vi "VIH Dialog - Quick Tips.vi"(10 "Tip#":i32=-1) -> (2 "Tip# out":i32=-1, 3 "ShowAtStartup out":bool)   [LabVIEW 2014]
doc: "::: VI Helpeks :::\nCopyright (c) 2000-2026 Konstantin Shifershteyn. All rights reserved."
uses:
  <vilib>/Platform/browser.llb/Open URL in Default Browser (string).vi
  _VIH Support Library.llb/VIH Utility - APP - Is Value Changed (U32).vi
  <vilib>/Utility/cursorutil.llb/Set Cursor (Icon Pict).vi
panel:
  out "counter":string
  in  "%First":bool
  out "Tip Title":string
  in  "%Next":bool
  in  "%Prev":bool
  in  "%OK":bool
  in  "ShowAtStartup":bool=TRUE caption="Don't show anymore"
  out "Tip Text":string
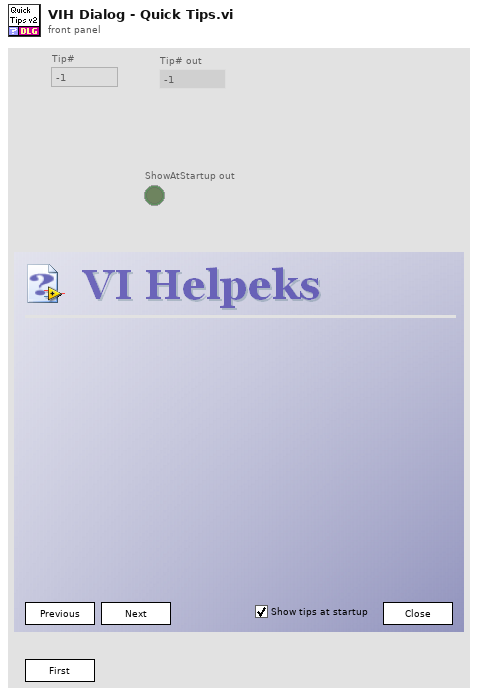
[diagram p1: front panel]
types:
  T1 = typedef "eventvkey.ctl" = enum16{"ASCII", "Enter", "Return", "Shift", "Ctrl", "Alt", "Cmd", "Opt", "Caps", "NumLock", "Clear", "Break", "Up", "Down", "Left", "Right", "Insert", "Delete", "Home", "End", "PageUp", "PageDown", "Escape", "Help", "Pause", "ScrollLock", "F1", "F2", "F3", "F4", "F5", "F6", "F7", "F8", "F9", "F10", "F11", "F12", "F13", "F14", "F15", "F16", "F17", "F18", "F19", "F20", "F21", "F22", "F23", "F24", "Play", "VolumeUp", "VolumeDown", "Mute", "Two Byte Char"}
  T2 = cluster{"Shift":bool, "Ctrl":bool, "Alt":bool, "Cmd":bool, "Opt":bool}
  T3 = typedef "LVPoint32TypeDef.ctl" = cluster{"Horizontal":i32, "Vertical":i32}
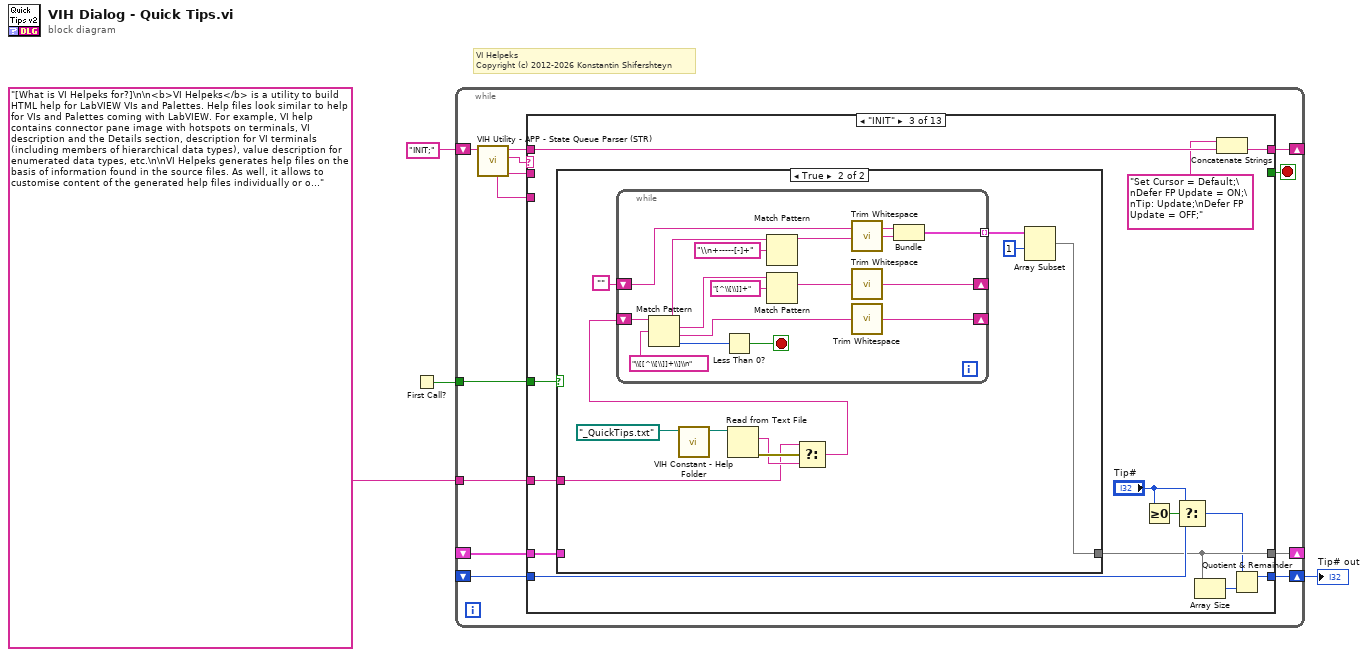
[diagram p0: block diagram]
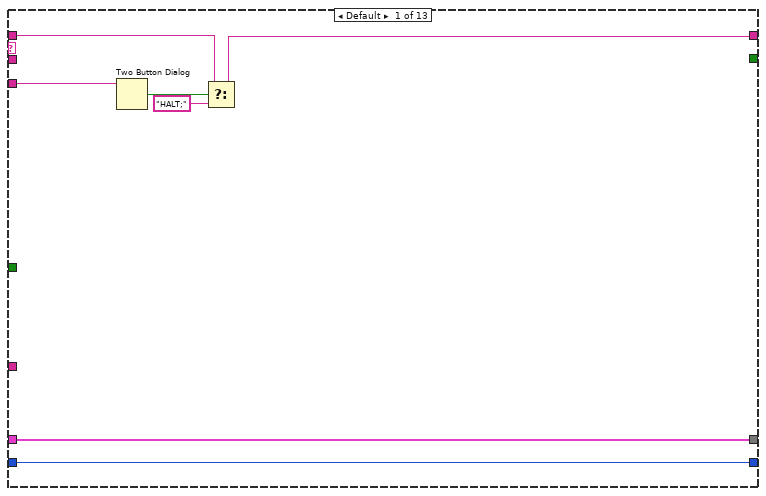
[diagram p2: hidden frame]
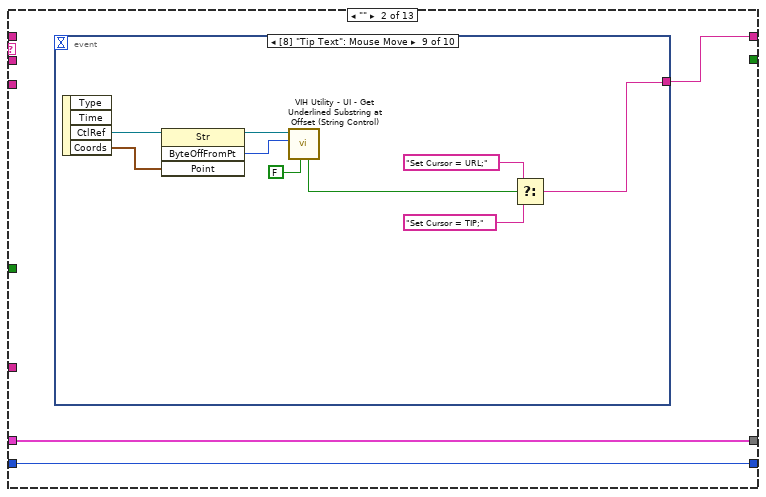
[diagram p3: hidden frame]
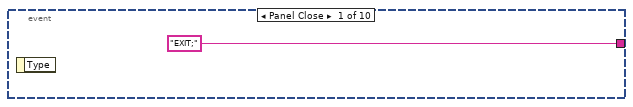
[diagram p4: hidden frame]
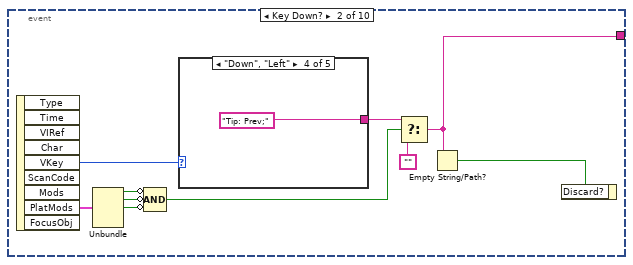
[diagram p5: hidden frame]
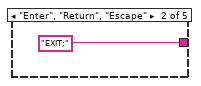
[diagram p7: hidden frame]
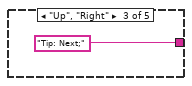
[diagram p8: hidden frame]
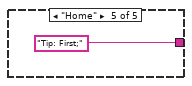
[diagram p9: hidden frame]
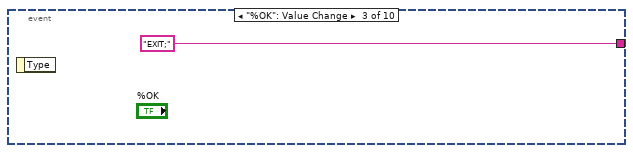
[diagram p10: hidden frame]
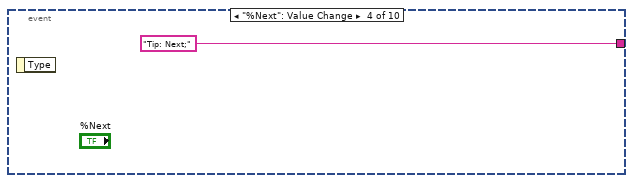
[diagram p11: hidden frame]
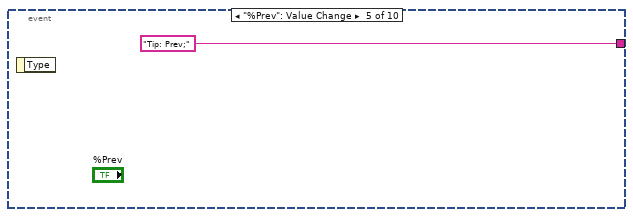
[diagram p12: hidden frame]
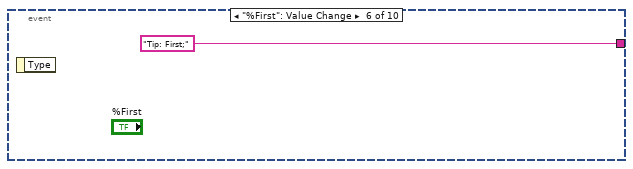
[diagram p13: hidden frame]
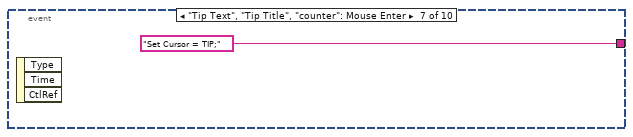
[diagram p14: hidden frame]
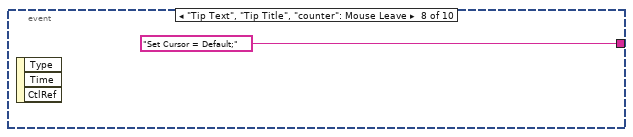
[diagram p15: hidden frame]
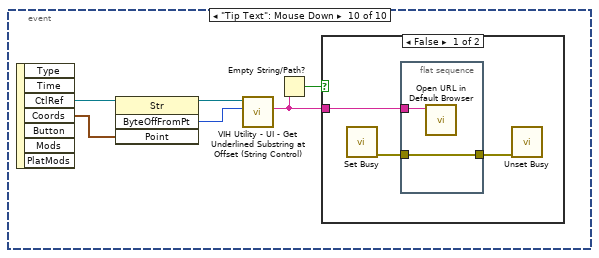
[diagram p16: hidden frame]
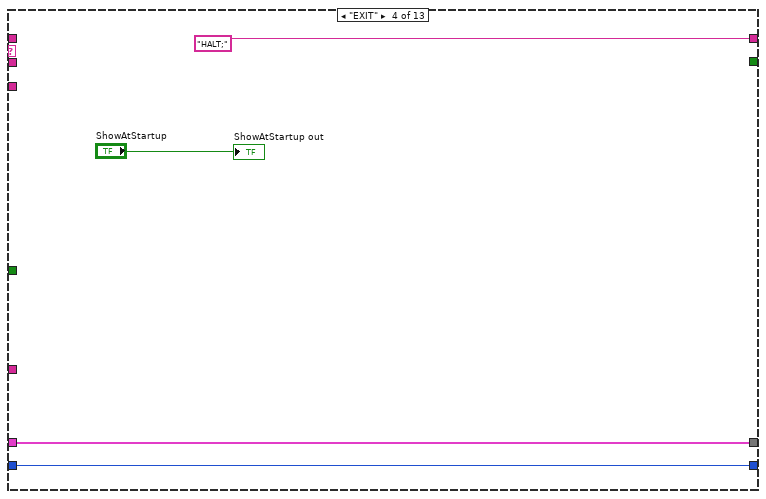
[diagram p19: hidden frame]
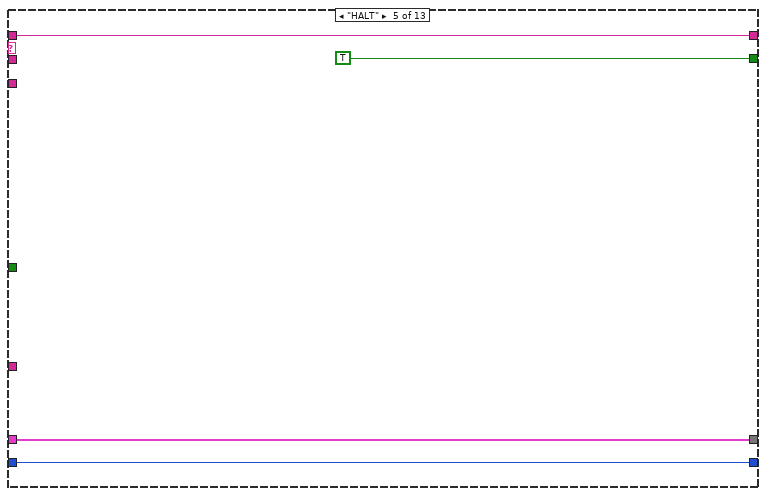
[diagram p20: hidden frame]
diagram:
  # "VI Helpeks\nCopyright (c) 2012-2026 Konstantin Shifershteyn"
  n1 = First Call?() -> (First Call?: T/F=w3:bool)
  n2 = while {
    shift-right: [w13] -> _
    shift-left: "INIT;" -> [w17]
    shift-right: [w11] -> _
    shift-left: _ -> [w10]
    shift-right: [w9] -> w1
    shift-left: _ -> [w8]
    tunnel: w3 -> [w7]
    tunnel: "[What is VI Helpeks for?]\n\n<b>VI Helpeks</b> is a utility to build HTML help for LabVIEW VIs and Palettes. Help files look similar to help for VIs and Palettes coming with LabVIEW. For example, VI help contains connector pane image with hotspots on terminals, VI description and the Details section, description for VI terminals (including members of hierarchical data types), value description for enumerated data types, etc.\n\nVI Helpeks generates help files on the basis of information found in the source files. As well, it allows to customise content of the generated help files individually or on group basis.\n\n------------------------\n\n[Help and Examples]\n\nTo learn overall concept of VI Helpeks, select <b>Help >> Open Help</b> menu.\n\nUse LabVIEW <b>Context Help</b> to get information on controls or indicators in the main VI Helpeks window as well as in any dialog. Context help might contain not only help on using a control or indicator but also relevant background information.\n\nVI Helpeks comes with a few example projects that demonstrate its capabilities and some details of use. Use <b>Help >> Open Example Project</b> menu to open an example project. When you open a project, build it with the <b>Build >> Build Help for All</b> menu. After the build completes, you can review generated help in your default browser.\n\n------------------------\n\n[A few GUI tips]\n\nShortcut menus are available for the Project Tree in the main VI Helpeks window as well as for controls in many dialog windows.\n\nMultiple items selection is allowed in tree and listbox controls in the main VI Helpeks window and dialog windows.\n\nYou can resize the main VI Helpeks window and some of dialog windows.\n\n------------------------\n\n[Build help]\n\nBuild help for all project files with <b>Build >> Build Help for All</b> menu.\n\nYou can build help for project files individually. For this, highlight desired file(s) in the Project Tree, activate shortcut menu and select either <b>Build Help (selected only)</b> or <b>Build Help (selected & underlying)</b>. The last option is for Palette menus, it will build help for the selected Palette and all its sub-palettes and VIs recursively.\n\nYou can build help for project files in a group. For this, highlight desired group(s) in the Project Tree, activate shortcut menu and select <b>Build help for underlying files</b>. Help will be built for all underlying files recursively.\n\n------------------------\n\n[Build Destination folder]\n\nWhen you create a new project or open an example project, destination folder for output files is set beneath the default temporary directory on your computer. If you want to change the target folder, select either <b>Help Project</b> or <b>Project Files</b> item in the Project Tree, select the <b>Target Paths</b> category and specify the desired path in the <b>Build Root Folder</b> control.\n\n------------------------\n\n[Open built help files]\n\nIn order to open an output help file, highlight the respective source file in the Project Tree, activate shortcut menu and select <b>Open Output Help File</b>. Also, you can do this using the main menu (<b>Project >> Open Output Help File</b>).\n\nVI Helpeks opens help files in your default browser.\n\n------------------------\n\n[Project types]\n\nVI Helpeks generates help files on the basis of template files. Appearance and behavior of output help files are defined by the set of template files used in a project. When you create a new project, its Master Rule is configured to use template files relevant for the project type you choose:\n*** <b>Default</b> project type is for generating pure frameless HTML files.\n*** <b>JavaScript based</b> project type is for generating HTML files that utilize JavaScripts for additional features.\n\nYou can easy reconfigure the Master Rule of your project for a desired project type through <b>File >> Change project type</b> menu.\n\n-----------------------\n\n[Images in help files]\n\nVI Helpeks creates help files with images that look the same as you see them in the LabVIEW version it's running. It does not use any template images for control terminals, but retrieves actual images from LabVIEW (including typedefs and members of hierarchical data structures). VI connector pane images look the same as in the LabVIEW Context Help.\n\n-----------------------\n\n[Hotspots in VI connector pane images]\n\nA help file generated for a VI contains connector pane image with hotspots at VI terminals. If you click a terminal name in the connector pane image, you are navigated to the respective control description in the help file.\n\nSimilarly, when you open <b>VI Terminals</b> dialog, you can click a VI terminal name in the connector pane image in order to select respective control (with its descendants, optionaly) in the Control Tree. Use Context Help for controls in this dialog to get more information.\n\n------------------------\n\n[Source VI state]\n\nSource VIs, for which you are going to build help, are not restricted to be in the idle state. VI Helpeks can build help for running VIs. As well, it can build help for locked and password protected VIs.\n\n------------------------\n\n[Compiled HTML Help (.CHM)]\n\nVI Helpeks doesn't create compiled help files (CHM) by itself. Instead, it creates HTML Help Project (HHP) for <b>HTML Help Workshop</b> by Microsoft, which can compile CHM files for you.\n\nSelect <b>Build >> Compiled HTML Help</b> menu to run a utility that helps you to create compiled help files.\n\nIf you don't have <b>HTML Help Workshop</b> installed, you can download it at Microsoft website for free:\n<link>http://msdn.microsoft.com/en-us/library/ms669985.aspx</link>\n" -> [w6]
    stop <- w12 stop-if-true
    n3 = call "VIH Utility - APP - State Queue Parser (STR).vi"("input queue"=w17) -> ("state parameters"=w5:string, "state"=w16:string, "remained queue"=w14:string, "complete state specifier"=w15:string)  [unwired: 5 in]
    n4 = case shown="\"INIT\"" w16 {
      tunnel: w15 -> [w24 _ _ _ _ _ _ _ _ _ _ _ _]
      tunnel: w14 -> [w22 _ w81 _ w116 w119 w127 w134 w142 w153 w161 w164 w174]
      tunnel: [w21 w27 w74 "HALT;" w116 w119 w127 w134 w142 w153 w155 w163 w173] -> w13
      tunnel: [_ _ _ _ TRUE _ _ _ _ _ _ _ _] -> w12
      tunnel: [w19 w26 w75 w110 w114 w118 w126 w133 w141 w146 w160 w171 w176] -> w11
      tunnel: w10 -> [w19 w26 w79 w110 w114 w118 w126 w133 w141 w146 w160 w171 w176]
      tunnel: [w18 w25 w70 w109 w113 w117 w125 w132 w140 w148 w158 w167 0] -> w9
      tunnel: w8 -> [w18 w25 w76 w109 w113 w117 w125 w132 w140 w148 w159 w170 _]
      tunnel: w7 -> [_ _ w80 _ _ _ _ _ _ _ _ _ _]
      tunnel: w6 -> [_ _ w78 _ _ _ _ _ _ _ _ _ _]
      tunnel: w5 -> [_ _ _ _ _ _ w120 w131 _ _ _ _ _]
      frame Default {
        n5 = Two Button Dialog(message=w24) -> (T button?=w23:bool)  [unwired: 2 in]
        n6 = Select(t=w22, s=w23, f="HALT;") -> (s? t:f=w21:string)
      }
      frame "" {
        n7 = event shown="[8] \"Tip Text\": Mouse Move" {
          selector: _ -> [_ _ _ _ _ _ _ _ _ _]
          dyn-events: _ -> [_ _ _ _ _ _ _ _ _ _]
          timeout: _ -> [_ _ _ _ _ _ _ _ _ _]
          tunnel: ["EXIT;" w30 "EXIT;" "Tip: Next;" "Tip: Prev;" "Tip: First;" "Set Cursor = TIP;" "Set Cursor = Default;" w53 _] -> w27
          event Panel Close {
            n8 = event-data() -> ()  [unwired: 1 in, 1 out]
          }
          event Key Down? {
            n9 = event-data() -> ("VKey"=w33:T1, "PlatMods"=w38:T2)  [unwired: 1 in, 7 out]
            n10 = Unbundle(w38) -> ("Shift"=w37:bool, "Ctrl"=w36:bool, "Alt"=w35:bool)  [unwired: 2 out]
            n11 = Compound Arithmetic op=AND(invert w37, invert w36, invert w35) -> (w34:bool)
            n12 = case shown="\"Down\", \"Left\"" w33 {
              tunnel: [_ "EXIT;" "Tip: Next;" "Tip: Prev;" "Tip: First;"] -> w32
              frame Default {
              }
              frame "Enter", "Return", "Escape" {
              }
              frame "Up", "Right" {
              }
              frame "Down", "Left" {
              }
              frame "Home" {
              }
            }
            n13 = Select(t=w32, s=w34, f="") -> (s? t:f=w30:string)
            n14 = Empty String/Path?(string/path=w30) -> (empty?=w31:bool)
            n15 = event-data("Discard?"=w31) -> ()  [unwired: 1 in, 1 out]
          }
          event "%OK": Value Change {
            n16 = event-data() -> ()  [unwired: 1 in, 1 out]
          }
          event "%Next": Value Change {
            n17 = event-data() -> ()  [unwired: 1 in, 1 out]
          }
          event "%Prev": Value Change {
            n18 = event-data() -> ()  [unwired: 1 in, 1 out]
          }
          event "%First": Value Change {
            n19 = event-data() -> ()  [unwired: 1 in, 1 out]
          }
          event "Tip Text", "Tip Title", "counter": Mouse Enter {
            n20 = event-data() -> ()  [unwired: 1 in, 3 out]
          }
          event "Tip Text", "Tip Title", "counter": Mouse Leave {
            n21 = event-data() -> ()  [unwired: 1 in, 3 out]
          }
          event "Tip Text": Mouse Move {
            n22 = event-data() -> ("CtlRef"=w56:refnum<vi>, "Coords"=w57:T3)  [unwired: 1 in, 2 out]
            n23 = invoke class="Str" method="ByteOffFromPt"(reference=w56, "Point"=w57) -> (reference out=w55:refnum<vi>, "ByteOffFromPt"=w54:i32)  [unwired: 2 in, 2 out]
            n24 = call "VIH Utility - UI - Get Underlined Substring at Offset (String Control).vi"("Get string (T)"=FALSE, "Offset"=w54, "Str Refnum"=w55) -> ("active"=w51:bool)  [unwired: 4 in, 4 out]
            n25 = Select(t="Set Cursor = URL;", s=w51, f="Set Cursor = TIP;") -> (s? t:f=w53:string)
          }
          event "Tip Text": Mouse Down {
            n26 = event-data() -> ("CtlRef"=w62:refnum<vi>, "Coords"=w63:T3)  [unwired: 1 in, 5 out]
            n27 = invoke class="Str" method="ByteOffFromPt"(reference=w62, "Point"=w63) -> (reference out=w61:refnum<vi>, "ByteOffFromPt"=w60:i32)  [unwired: 2 in, 2 out]
            n28 = call "VIH Utility - UI - Get Underlined Substring at Offset (String Control).vi"("Offset"=w60, "Str Refnum"=w61) -> ("String"=w59:string)  [unwired: 5 in, 4 out]
            n29 = Empty String/Path?(string/path=w59) -> (empty?=w58:bool)
            n30 = case shown="False" w58 {
              tunnel: w59 -> [w66 _]
              frame False {
                n31 = call <vilib>:"Set Busy.vi"() -> ("error out"=w64:errorcluster)  [unwired: 10 in, 1 out]
                n32 = flat-sequence {
                  tunnel: w66 -> [w68]
                  tunnel: [w67] -> w65
                  tunnel: w64 -> [w67]
                  frame #0 {
                    n33 = call-poly <vilib>:"Open URL in Default Browser.vi"("URL"=w68) -> ()  [unwired: 5 in, 2 out]
                  }
                }
                n34 = call <vilib>:"Unset Busy.vi"("error in (no error)"=w65) -> ()  [unwired: 10 in, 1 out]
              }
              frame True {
              }
            }
          }
        }
      }
      frame "INIT" {
        n35 = case shown="True" w80 {
          tunnel: [w82 w85] -> w75
          tunnel: w79 -> [w82 _]
          tunnel: w78 -> [_ w87]
          frame False {
          }
          frame True {
            n36 = call "VIH Constant - Help Folder.vi"("append path"=path "_QuickTips.txt" ("Path")) -> ("Help path"=w84:path)  [unwired: 10 in]
            n37 = Read from Text File(file (use dialog)=w84) -> (text=w88:string, error out=w89:errorcluster)  [unwired: 3 in, 2 out]
            n38 = Select(t=w87, s=w89, f=w88) -> (s? t:f=w86:string)
            n39 = while {
              shift-right: [w97] -> _
              shift-left: w86 -> [w108]
              shift-right: [w98] -> _
              shift-left: "" -> [w101]
              tunnel: [w100] -> w91 mode=indexing
              stop <- w105 stop-if-true
              n40 = Match Pattern(string=w108, regular expression="\\[[^\\[\\]]+\\]\\n") -> (before substring=w93:string, match substring=w95:string, after substring=w104:string, offset past match=w106:i32)  [unwired: 1 in]
              n41 = Less Than 0?(x=w106) -> (x < 0?=w105:bool)
              n42 = Match Pattern(string=w93, regular expression="\\n+-----[-]+") -> (before substring=w94:string)  [unwired: 1 in, 3 out]
              n43 = Match Pattern(string=w95, regular expression="[^\\[\\]]+") -> (match substring=w102:string)  [unwired: 1 in, 3 out]
              n44 = call <vilib>:"Trim Whitespace.vi"("string"=w94) -> ("trimmed string"=w99:string)  [unwired: 1 in]
              n45 = call <vilib>:"Trim Whitespace.vi"("string"=w102) -> ("trimmed string"=w98:string)  [unwired: 1 in]
              n46 = call <vilib>:"Trim Whitespace.vi"("string"=w104) -> ("trimmed string"=w97:string)  [unwired: 1 in]
              n47 = Bundle(w101, "trimmed string"=w99) -> (w100:cluster{string, "trimmed string":string})  [unwired: 1 in]
            }
            n48 = Array Subset(array=w91, index=1) -> (w85:cluster{string, "trimmed string":string}[])  [unwired: 1 in]
          }
        }
        n49 = Greater Or Equal To 0?(x="Tip#") -> (x >= 0?=w77:bool)
        n50 = Select(t="Tip#", s=w77, f=w76) -> (s? t:f=w69:i32)
        n51 = Array Size(array=w75) -> (size(s)=w71:i32)
        n52 = Concatenate Strings("Set Cursor = Default;\nDefer FP Update = ON;\nTip: Update;\nDefer FP Update = OFF;", w81) -> (w74:string)
        n53 = Quotient & Remainder(x=w69, y=w71) -> (x-y*floor(x/y)=w70:i32)  [unwired: 1 out]
      }
      frame "EXIT" {
        "ShowAtStartup out" <- "ShowAtStartup"
      }
      frame "HALT" {
      }
      frame "------------------------------ 1" {
      }
      frame "Defer FP Update" {
        n54 = To Upper Case(1:w120) -> (0:w123:string)
        n55 = Equal?(x=w123, y="ON") -> (x = y?=w121:bool)
        n56 = property class="VI"() -> ("Panel"=w124:refnum<vi>)  [unwired: 2 in, 2 out]
        n57 = property class="Pnl"(reference=w124, "DeferPanUpdts"=w121) -> ()  [unwired: 1 in, 2 out]
      }
      frame "Set Cursor" {
        n58 = case shown="\"Default\", Default" w131 {
          tunnel: [u16 6 ("icon") u16 1 ("icon") u16 6 ("icon")] -> w130
          tunnel: [_ _ TRUE] -> _
          frame "Default", Default {
          }
          frame "TIP" {
          }
          frame "URL" {
          }
        }
        n59 = To Unsigned Long Integer(number=w130) -> (unsigned 32bit integer=w129:u32)
        n60 = call-poly "VIH Utility - APP - Is Value Changed.vi"("Value"=w129) -> ("Changed"=w128:bool)  [unwired: 5 in, 1 out]
        n61 = case shown="True" w128 {
          tunnel: w130 -> [_ w135]
          frame False {
          }
          frame True {
            n62 = call-poly <vilib>:"Set Cursor.vi"("icon"=w135) -> ()  [unwired: 9 in, 2 out]
          }
        }
      }
      frame "------------------------------ 2" {
      }
      frame "Tip: Update" {
        n63 = Index Array(array=w146, index=w148) -> (element=w152:cluster{string, "trimmed string":string})
        n64 = Unbundle(w152) -> (→"Tip Title":string, "trimmed string"=w143:string)
        n65 = Array Size(array=w146) -> (size(s)=w145:i32)
        n66 = Increment(x=w148) -> (x+1=w147:i32)
        n67 = Format Into String(format string="Tip %d of %d", w147, w145) -> (resulting string=→"counter":string)  [unwired: 2 in, 1 out]
        n68 = control-ref of="Tip Text"() -> (w144:refnum<vi>)
        n69 = call "VIH Utility - UI - Display Formatted Text (String Control).vi"("Formatted text"=w143, "Str Refnum"=w144) -> ()  [unwired: 8 in, 2 out]
      }
      frame "Tip: Next" {
        n70 = Increment(x=w159) -> (x+1=w157:i32)
        n71 = Array Size(array=w160) -> (size(s)=w156:i32)
        n72 = Quotient & Remainder(x=w157, y=w156) -> (x-y*floor(x/y)=w158:i32)  [unwired: 1 out]
        n73 = Concatenate Strings("Defer FP Update = ON;\nTip: Update;\nDefer FP Update = OFF;", w161) -> (w155:string)
      }
      frame "Tip: Prev" {
        n74 = Array Size(array=w171) -> (size(s)=w166:i32)
        n75 = Decrement(x=w170) -> (x-1=w169:i32)
        n76 = Decrement(x=w166) -> (x-1=w165:i32)
        n77 = Less Than 0?(x=w169) -> (x < 0?=w168:bool)
        n78 = Select(t=w165, s=w168, f=w169) -> (s? t:f=w167:i32)
        n79 = Concatenate Strings("Defer FP Update = ON;\nTip: Update;\nDefer FP Update = OFF;", w164) -> (w163:string)
      }
      frame "Tip: First" {
        n80 = Concatenate Strings("Defer FP Update = ON;\nTip: Update;\nDefer FP Update = OFF;", w174) -> (w173:string)
      }
    }
  }
  "Tip# out" <- w1
